vi "SA mark Harmonic Frequency.vi"(8 "error in (no error)":errorcluster caption="에러 입력(에러 없음)", 9 "Frequency":dbl[](array[numeric]), 10 "isExceed?":bool[](array[boolean]), 11 "Instrument Manager 입력":refnum<class "Instrument Manager.lvclass">) -> (0 "error out":errorcluster caption="에러 출력", 3 "Instrument Manager 출력":refnum<class "Instrument Manager.lvclass">)   [LabVIEW 2023, in "Instrument Manager.lvclass"]
uses:
  Instrument Manager.lvclass
  Instrument Manager.lvclass/Instrument Manager.ctl
  Module/Spectrum Analyzer/Interface_Spectrum/Interface_Spectrum.lvclass
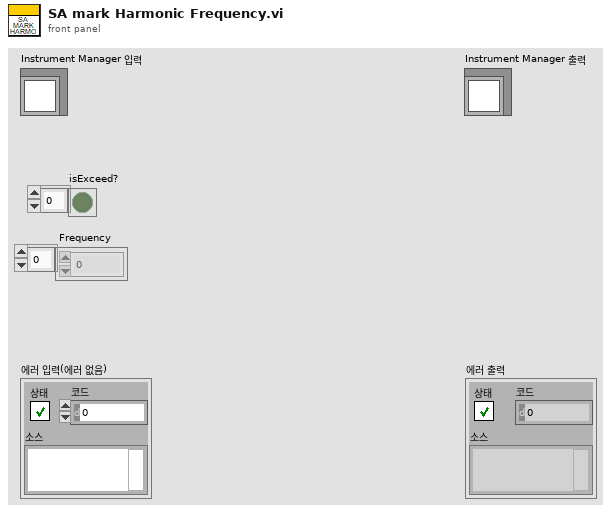
[diagram p1: front panel]
types:
  T1 = cluster{"Anritsu Call Box":refnum<class "Anritsu Call Box.lvclass">, "Spectrum Analyzer":refnum<class "Interface_Spectrum.lvclass">, "RF Switch Box":refnum<class "RF Filter Box.lvclass">, "Turn Table":refnum<class "Interface - Turn Table.lvclass">, "Mast":refnum<class "Interface - Mast.lvclass">, "3D Controller":refnum<class "Interface_3D Controller.lvclass">}
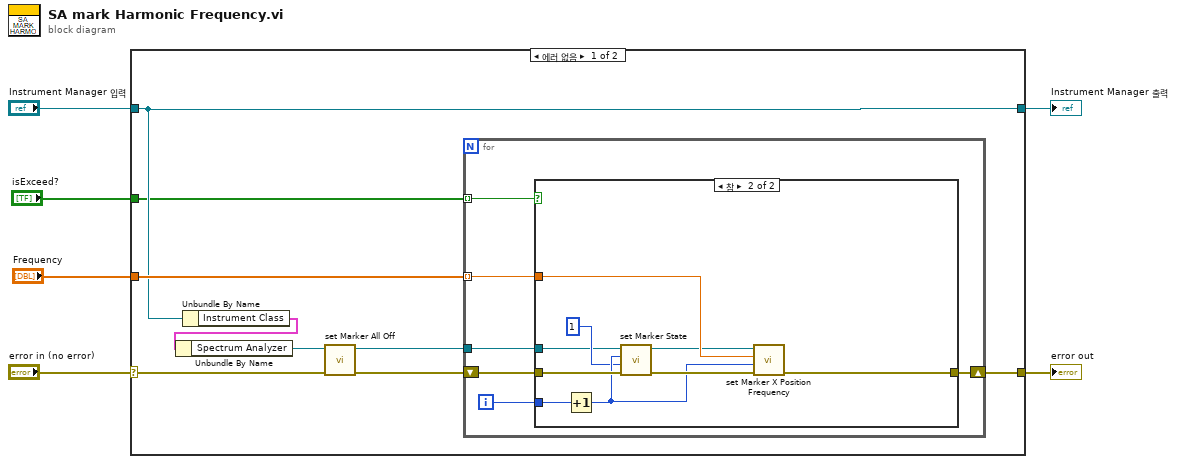
[diagram p0: block diagram]
diagram:
  n1 = case shown="에러 없음" "error in (no error)" {
    selector: "error in (no error)" -> [w9 w33]
    tunnel: [w15 w33] -> w5
    tunnel: [w12 w32] -> w3
    tunnel: "Instrument Manager 입력" -> [w12 w32]
    tunnel: "isExceed?" -> [w11 _]
    tunnel: "Frequency" -> [w14 _]
    frame No Error {
      n2 = Unbundle By Name(w12) -> ("Instrument Class"=w13:T1)
      n3 = Unbundle By Name(w13) -> ("Spectrum Analyzer"=w10:refnum<class "Interface_Spectrum.lvclass">)
      n4 = call-dynamic "set Marker All Off.vi"("error in (no error)"=w9, "Interface_Spectrum in"=w10) -> ("error out"=w7:errorcluster, "Interface_Spectrum out"=w8:refnum<class "Interface_Spectrum.lvclass">)  [unwired: 8 in]
      n5 = for {
        tunnel: w11 -> [w21] mode=indexing
        tunnel: w14 -> [w18] mode=indexing
        shift-right: [w19] -> w15
        shift-left: w7 -> [w17]
        tunnel: w8 -> [w16]
        i -> [w20]
        n6 = case shown="참" w21 {
          tunnel: w17 -> [w22 w30]
          tunnel: w20 -> [_ w31]
          tunnel: [w22 w28] -> w19
          tunnel: w18 -> [_ w27]
          tunnel: w16 -> [_ w24]
          frame False {
          }
          frame True {
            n7 = Increment(x=w31) -> (x+1=w26:i32)
            n8 = call-dynamic "set Marker State.vi"("error in (no error)"=w30, "trace index"=1, "Marker Index"=w26, "Interface_Spectrum in"=w24) -> ("error out"=w29:errorcluster, "Interface_Spectrum out"=w23:refnum<class "Interface_Spectrum.lvclass">)  [unwired: 6 in]
            n9 = call-dynamic "set Marker X Position Frequency.vi"("error in (no error)"=w29, "Index"=w26, "X Position Frequency (Hz)"=w27, "Interface_Spectrum in"=w23) -> ("error out"=w28:errorcluster)  [unwired: 6 in, 1 out]
          }
        }
      }
    }
    frame Error {
    }
  }
  "error out" <- w5
  "Instrument Manager 출력" <- w3
